vi "get_ACS_status.vi"() -> ()   [LabVIEW 2018]
uses:
  RxTx/RxTx.lvclass
  <vilib>/addons/zeromq/socket_type.ctl
  <vilib>/addons/zeromq/socket_options.ctl
  <vilib>/addons/zeromq/zmq_socket.lvclass
  <vilib>/addons/zeromq/zmq_context.lvclass
  <vilib>/addons/zeromq/zeromq.lvlib
panel:
  in  "RxTx in 2":refnum<class "RxTx.lvclass">
  in  "RxTx in":refnum<class "RxTx.lvclass">
  in  "Stop Button":bool
  out "error out":errorcluster
  out "error out 3":errorcluster
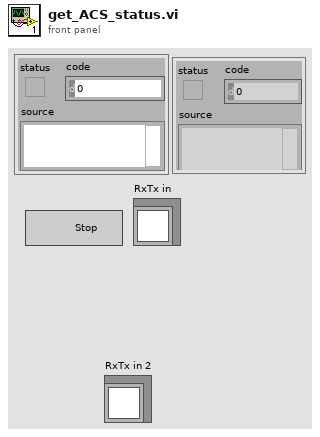
[diagram p1: front panel]
types:
  T1 = typedef "zeromq.lvlib/socket_options.ctl" = enum8{"NONE", "ZMQ_HWM", "<2>", "ZMQ_SWAP", "ZMQ_AFFINITY", "ZMQ_ROUTING_ID", "ZMQ_SUBSCRIBE", "ZMQ_UNSUBSCRIBE", "ZMQ_RATE", "ZMQ_RECOVERY_IVL", "ZMQ_MCAST_LOOP", "ZMQ_SNDBUF", "ZMQ_RCVBUF", "ZMQ_RCVMORE", "ZMQ_FD", "ZMQ_EVENTS", "ZMQ_TYPE", "ZMQ_LINGER", "ZMQ_RECONNECT_IVL", "ZMQ_BACKLOG", "ZMQ_RECOVERY_IVL_MSEC", "ZMQ_RECONNECT_IVL_MAX", "ZMQ_MAXMSGSIZE", "ZMQ_SNDHWM", "ZMQ_RCVHWM", "ZMQ_MULTICAST_HOPS", "<26>", "ZMQ_RCVTIMEO", "ZMQ_SNDTIMEO", "<29>", "<30>", "ZMQ_IPV4ONLY", "ZMQ_LAST_ENDPOINT", "ZMQ_ROUTER_MANDATORY", "ZMQ_TCP_KEEPALIVE", "ZMQ_TCP_KEEPALIVE_CNT", "ZMQ_TCP_KEEPALIVE_IDLE", "ZMQ_TCP_KEEPALIVE_INTVL", "ZMQ_TCP_ACCEPT_FILTER", "ZMQ_IMMEDIATE", "ZMQ_XPUB_VERBOSE", "ZMQ_ROUTER_RAW", "ZMQ_IPV6", "ZMQ_MECHANISM", "ZMQ_PLAIN_SERVER", "ZMQ_PLAIN_USERNAME", "ZMQ_PLAIN_PASSWORD", "ZMQ_CURVE_SERVER", "ZMQ_CURVE_PUBLICKEY", "ZMQ_CURVE_SECRETKEY", "ZMQ_CURVE_SERVERKEY", "ZMQ_PROBE_ROUTER", "ZMQ_REQ_CORRELATE", "ZMQ_REQ_RELAXED", "ZMQ_CONFLATE", "ZMQ_ZAP_DOMAIN", "ZMQ_ROUTER_HANDOVER", "ZMQ_TOS", "ZMQ_IPC_FILTER_PID", "ZMQ_IPC_FILTER_UID", "ZMQ_IPC_FILTER_GID", "ZMQ_CONNECT_ROUTING_ID", "ZMQ_GSSAPI_SERVER", "ZMQ_GSSAPI_PRINCIPAL", "ZMQ_GSSAPI_SERVICE_PRINCIPAL", "ZMQ_GSSAPI_PLAINTEXT", "ZMQ_HANDSHAKE_IVL", "<67>", "ZMQ_SOCKS_PROXY", "ZMQ_XPUB_NODROP", "ZMQ_BLOCKY", "ZMQ_XPUB_MANUAL", "ZMQ_XPUB_WELCOME_MSG", "ZMQ_STREAM_NOTIFY", "ZMQ_INVERT_MATCHING", "ZMQ_HEARTBEAT_IVL", "ZMQ_HEARTBEAT_TTL", "ZMQ_HEARTBEAT_TIMEOUT", "ZMQ_XPUB_VERBOSER", "ZMQ_CONNECT_TIMEOUT", "ZMQ_TCP_MAXRT", "ZMQ_THREAD_SAFE", "<82>", "<83>", "ZMQ_MULTICAST_MAXTPDU", "ZMQ_VMCI_BUFFER_SIZE", "ZMQ_VMCI_BUFFER_MIN_SIZE", "ZMQ_VMCI_BUFFER_MAX_SIZE", "ZMQ_VMCI_CONNECT_TIMEOUT", "ZMQ_USE_FD", "ZMQ_GSSAPI_PRINCIPAL_NAMETYPE", "ZMQ_GSSAPI_SERVICE_PRINCIPAL_NAMETYPE", "ZMQ_BINDTODEVICE", "ZMQ_ZAP_ENFORCE_DOMAIN", "ZMQ_LOOPBACK_FASTPATH", "ZMQ_METADATA", "ZMQ_MULTICAST_LOOP", "ZMQ_ROUTER_NOTIFY"}
  T2 = typedef "zeromq.lvlib/socket_type.ctl" = enum8{"ZMQ_PAIR", "ZMQ_PUB", "ZMQ_SUB", "ZMQ_REQ", "ZMQ_REP", "ZMQ_DEALER", "ZMQ_ROUTER", "ZMQ_PULL", "ZMQ_PUSH", "ZMQ_XPUB", "ZMQ_XSUB", "ZMQ_STREAM", "ZMQ_SERVER", "ZMQ_CLIENT", "ZMQ_RADIO", "ZMQ_DISH", "ZMQ_GATHER", "ZMQ_SCATTER", "ZMQ_DGRAM"}
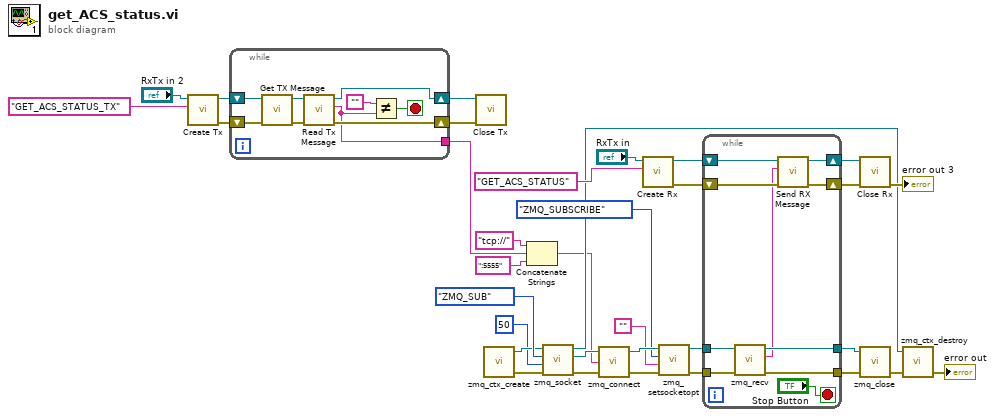
[diagram p0: block diagram]
diagram:
  n1 = call "Create Tx.vi"("Writer Name"="GET_ACS_STATUS_TX", "RxTx in"="RxTx in 2") -> ("error out"=w4:errorcluster, "RxTx out"=w5:refnum<class "RxTx.lvclass">)  [unwired: 8 in]
  n2 = while {
    shift-right: [w36] -> w3
    shift-left: w4 -> [w41]
    shift-right: [w37] -> w2
    shift-left: w5 -> [w40]
    tunnel: [w35] -> w1
    stop <- w42 stop-if-true
    n3 = call "Get TX Message.vi"("error in (no error)"=w41, "RxTx in"=w40) -> ("error out"=w39:errorcluster, "RxTx out"=w38:refnum<class "RxTx.lvclass">)  [unwired: 8 in]
    n4 = call "Read Tx Message.vi"("error in (no error)"=w39, "RxTx in"=w38) -> ("error out"=w36:errorcluster, "Tx Message"=w35:string, "RxTx out"=w37:refnum<class "RxTx.lvclass">)  [unwired: 7 in]
    n5 = Not Equal?(x="", y=w35) -> (x != y?=w42:bool)
  }
  n6 = call "Close Tx.vi"("error in (no error)"=w3, "RxTx in"=w2) -> ()  [unwired: 8 in, 2 out]
  n7 = call <vilib>:"zmq_ctx_create.vi"() -> ("error out"=w24:errorcluster, "context out"=w17:refnum<class "zmq_context.lvclass">)  [unwired: 4 in]
  n8 = Concatenate Strings("tcp://" ("endpoint"), w1, ":5555" ("endpoint")) -> (w10:string)
  n9 = call <vilib>:"zmq_socket.vi"("error in"=w24, "linger (ms)"=50, "socket type"=socket_type."ZMQ_SUB", "context in"=w17) -> ("error out"=w23:errorcluster, "socket out"=w18:refnum<class "zmq_socket.lvclass">, "context out"=w13:refnum<class "zmq_context.lvclass">)  [unwired: 1 in]
  n10 = call <vilib>:"zmq_connect.vi"("error in"=w23, "endpoint"=w10, "socket in"=w18) -> ("error out"=w21:errorcluster, "socket out"=w22:refnum<class "zmq_socket.lvclass">)  [unwired: 1 in]
  n11 = call "Create Rx.vi"("Reader Name"="GET_ACS_STATUS" ("Writer Name"), "RxTx in"="RxTx in") -> ("error out"=w9:errorcluster, "RxTx out"=w8:refnum<class "RxTx.lvclass">)  [unwired: 8 in]
  n12 = call <vilib>:"zmq_setsocketopt.vi"("error in"=w21, "value"="", "option"=socket_options."ZMQ_SUBSCRIBE", "socket in"=w22) -> ("error out"=w15:errorcluster, "socket out"=w14:refnum<class "zmq_socket.lvclass">)  [unwired: 2 in]
  n13 = while {
    shift-right: [w45] -> w29
    shift-left: w8 -> [w47]
    shift-right: [w44] -> w28
    shift-left: w9 -> [w48]
    tunnel: w14 -> [w53]
    tunnel: w15 -> [w52]
    tunnel: [w51] -> w33
    tunnel: [w50] -> w32
    stop <- "Stop Button" stop-if-true
    n14 = call <vilib>:"zmq_recv.vi"("error in"=w52, "socket in"=w53) -> ("error out"=w50:errorcluster, "data"=w46:string, "socket out"=w51:refnum<class "zmq_socket.lvclass">)  [unwired: 3 in, 2 out]
    n15 = call "Send RX Message.vi"("error in (no error)"=w48, "message"=w46, "RxTx in"=w47) -> ("error out"=w44:errorcluster, "RxTx out"=w45:refnum<class "RxTx.lvclass">)  [unwired: 7 in]
  }
  n16 = call "Close Rx.vi"("error in (no error)"=w28, "RxTx in"=w29) -> ("error out"=→"error out 3":errorcluster)  [unwired: 8 in, 1 out]
  n17 = call <vilib>:"zmq_close.vi"("error in"=w32, "socket"=w33) -> ("error out"=w34:errorcluster)  [unwired: 3 in]
  n18 = call <vilib>:"zmq_ctx_destroy.vi"("error in"=w34, "context in"=w13) -> ("error out"=→"error out":errorcluster)  [unwired: 3 in]
